vi "Module ID.vi"(11 "Module in":refnum<class "Module.lvclass">) -> (2 "Module ID":string)   [LabVIEW 2020, in "Volatus.lvlib" / "Module.lvclass"]
uses:
  Module.lvclass
  Module.lvclass/Module.ctl
  VolatusConfig/VolatusConfigElement/VolatusConfigElement.lvclass
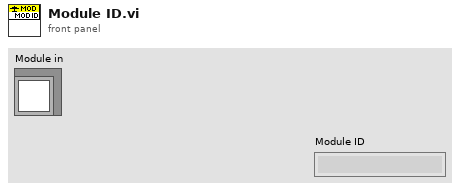
[diagram p1: front panel]
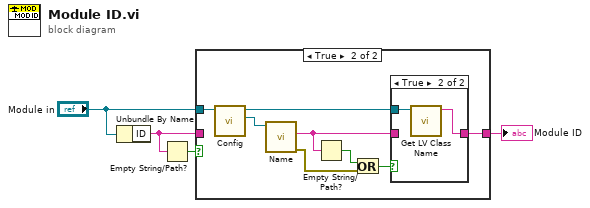
[diagram p0: block diagram]
diagram:
  n1 = Unbundle By Name("Module in") -> ("ID"=w3:string)
  n2 = Empty String/Path?(string/path=w3) -> (empty?=w4:bool)
  n3 = case shown="True" w4 {
    tunnel: w3 -> [w5 _]
    tunnel: "Module in" -> [_ w12]
    tunnel: [w5 w7] -> w2
    frame False {
    }
    frame True {
      n4 = call "Config.vi"("Module in"=w12) -> ("Config"=w13:refnum<class "VolatusConfigElement.lvclass">, "Module out"=w8:refnum<class "Module.lvclass">)  [unwired: 9 in]
      n5 = call "Name.vi"("VolatusConfigElement in"=w13) -> ("error out"=w11:errorcluster, "Name"=w6:string)  [unwired: 8 in, 1 out]
      n6 = Empty String/Path?(string/path=w6) -> (empty?=w10:bool)
      n7 = Or(x=w10, y=w11) -> (x .or. y?=w9:bool)
      n8 = case shown="True" w9 {
        tunnel: w8 -> [_ w16]
        tunnel: [w14 w15] -> w7
        tunnel: w6 -> [w14 _]
        frame False {
        }
        frame True {
          n9 = call <vilib>:"Get LV Class Name.vi"("object"=w16) -> ("class name"=w15:string)  [unwired: 9 in, 1 out]
        }
      }
    }
  }
  "Module ID" <- w2
